vi "提示等待.vi"() -> (0 "error out":errorcluster caption="错误输出")   [LabVIEW 2025]
uses:
  global.vi
panel:
  in  "文本":string="等待工具换钉，更换后请按启动键继续进行测试；\n如取消测试，请按停止键。"
  in  "继续":bool
  in  "停止":bool
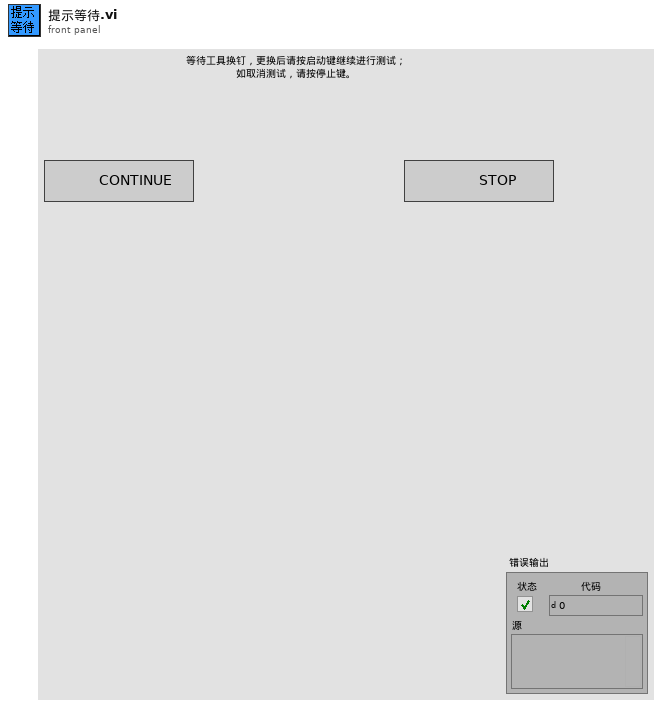
[diagram p1: front panel]
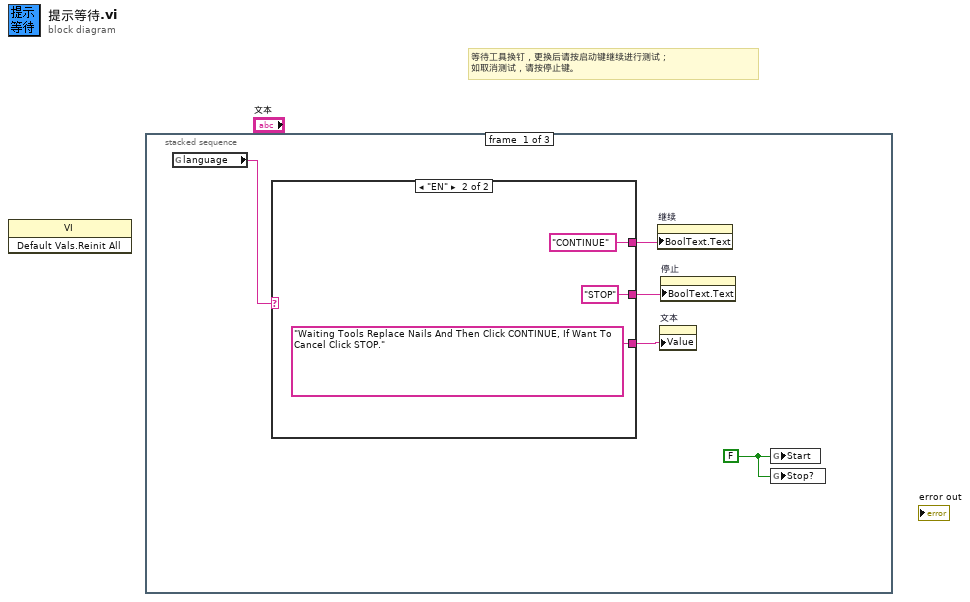
[diagram p0: block diagram]
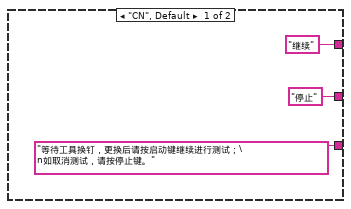
[diagram p2: hidden frame]
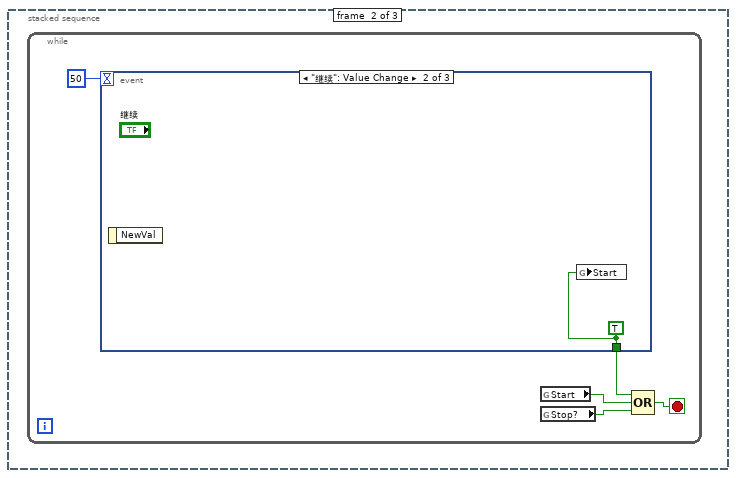
[diagram p3: hidden frame]
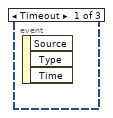
[diagram p4: hidden frame]
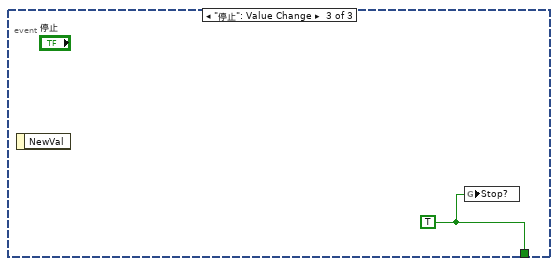
[diagram p5: hidden frame]
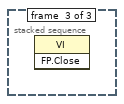
[diagram p6: hidden frame]
diagram:
  # "等待工具换钉，更换后请按启动键继续进行测试；\n如取消测试，请按停止键。"
  n1 = invoke class="VI" method="Default Vals.Reinit All"() -> ()  [unwired: 3 in, 3 out]
  n2 = stacked-sequence {
    frame #0 {
      w5 = FALSE ("Start")
      n3 = global read "global.vi" "language"() -> (w4:string)
      n4 = case shown="\"EN\"" w4 {
        tunnel: ["继续" "CONTINUE"] -> w3
        tunnel: ["停止" "STOP"] -> w2
        tunnel: ["等待工具换钉，更换后请按启动键继续进行测试；\n如取消测试，请按停止键。" "Waiting Tools Replace Nails And Then Click CONTINUE, If Want To Cancel Click STOP."] -> w1
        frame "CN", Default {
        }
        frame "EN" {
        }
      }
      n5 = property on="继续" class="Bool"("BoolText.Text"=w3) -> ()  [unwired: 2 in, 2 out]
      n6 = property on="文本" class="Str"("Value"=w1) -> ()  [unwired: 2 in, 2 out]
      n7 = property on="停止" class="Bool"("BoolText.Text"=w2) -> ()  [unwired: 2 in, 2 out]
      n8 = global write "global.vi" "Start"(w5) -> ()
      n9 = global write "global.vi" "Stop?"(w5) -> ()
    }
    frame #1 {
      n10 = while {
        stop <- w16 stop-if-true
        n11 = event shown="[1] \"继续\": Value Change" {
          selector: _ -> [_ _ _]
          dyn-events: _ -> [_ _ _]
          timeout: 50 -> [_ _ _]
          tunnel: [_ w17 w18] -> w12
          event Timeout {
            n12 = event-data() -> ()  [unwired: 1 in, 3 out]
          }
          event "继续": Value Change {
            w17 = TRUE
            n13 = event-data() -> ()  [unwired: 1 in, 1 out]
            n14 = global write "global.vi" "Start"(w17) -> ()
          }
          event "停止": Value Change {
            w18 = TRUE
            n15 = event-data() -> ()  [unwired: 1 in, 1 out]
            n16 = global write "global.vi" "Stop?"(w18) -> ()
          }
        }
        n17 = global read "global.vi" "Start"() -> (w15:bool)
        n18 = global read "global.vi" "Stop?"() -> (w13:bool)
        n19 = Compound Arithmetic op=OR(w12, w15, w13) -> (w16:bool)
      }
    }
    frame #2 {
      n20 = invoke class="VI" method="FP.Close"() -> ()  [unwired: 3 in, 3 out]
    }
  }
